vi "GOOP_ClassTemplateLookup.vi"(10 "ClassType":string, 11 "ClassTemplateFolderIn":path) -> (3 "ClassTemplateFolderOut":path)   [LabVIEW 2020]
uses:
  <vilib>/Utility/config.llb/Read Key (Path).vi
  <vilib>/Utility/config.llb/NI_LVConfig.lvlib
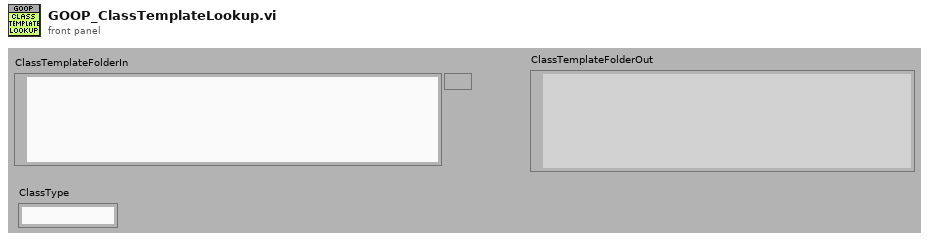
[diagram p1: front panel]
types:
  T1 = typedef "NI_LVConfig.lvlib/Config Data RefNum.ctl" = refnum<k1>
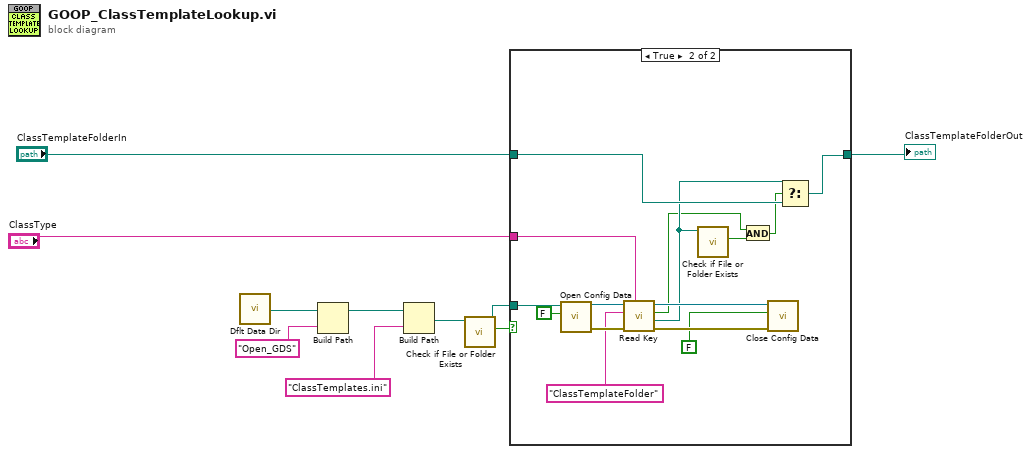
[diagram p0: block diagram]
diagram:
  n1 = call <vilib>:"Dflt Data Dir.vi"() -> ("App:Default Data Directory"=w10:path)
  n2 = Build Path(base path=w10, name or relative path="Open_GDS") -> (appended path=w8:path)
  n3 = Build Path(base path=w8, name or relative path="ClassTemplates.ini") -> (appended path=w6:path)
  n4 = call <vilib>:"Check if File or Folder Exists.vi"("path"=w6) -> ("file or folder exists?"=w5:bool, "dup path"=w4:path)  [unwired: 8 in, 1 out]
  n5 = case shown="True" w5 {
    tunnel: w4 -> [_ w23]
    tunnel: "ClassType" -> [_ w22]
    tunnel: "ClassTemplateFolderIn" -> [w11 w18]
    tunnel: [w11 w17] -> w1
    frame False {
    }
    frame True {
      n6 = call <vilib>:"Open Config Data.vi"("create file if necessary (T)"=FALSE, "configuration file path"=w23) -> ("error out"=w25:errorcluster, "refnum"=w26:T1)  [unwired: 7 in, 1 out]
      n7 = call-poly <vilib>:"Read Key.vi"("section"=w22, "error in (no error)"=w25, "key"="ClassTemplateFolder", "refnum"=w26) -> ("error out"=w19:errorcluster, "value"=w15:path, "found?"=w13:bool, "refnum out"=w20:T1)  [unwired: 4 in]
      n8 = call <vilib>:"Check if File or Folder Exists.vi"("path"=w15) -> ("file or folder exists?"=w14:bool)  [unwired: 8 in, 2 out]
      n9 = And(x=w13, y=w14) -> (x .and. y?=w12:bool)
      n10 = call <vilib>:"Close Config Data.vi"("error in (no error)"=w19, "write file if changed (T)"=FALSE ("create file if necessary (T)"), "refnum"=w20) -> ()  [unwired: 7 in, 2 out]
      n11 = Select(t=w15, s=w12, f=w18) -> (s? t:f=w17:path)
    }
  }
  "ClassTemplateFolderOut" <- w1
